vi "Smart_Elevator_TCP.vi"() -> ()   [LabVIEW 2026]
uses:
  Projet_labview/Control 5.ctl
  Projet_labview/Control 6.ctl
  Projet_labview/Control 1.ctl
  <vilib>/Utility/miscctls.llb/LVPositionTypeDef.ctl
panel:
  out "TCP Command Code":i32
  out "Boolean 2":bool
  out "Boolean":bool=TRUE
  out "Numeric 3":i32=2
  out "Numeric 2":i32=1
  out "Numeric":i32
  out "Received Commad":string
  out "?":bool
  out "?":bool
  out "?":picture
  out "Elevator Position":dbl(slide) scale=0.0..2.0 scale format="%#.1g"
  in  "Reset":bool
  out "Curent_STATE":T1
  in  "Quitter":bool
  in  "Urgence_button":bool
  in  "Floor_2":bool
  in  "Floor_1":bool
  in  "RDC":bool
  out "Elevator_STATUS":T3
  # "SMART ELEVATOR CONTROL"
  # "INTELLIGENT LIFT MONITORING & CONTROL"
  # "Elevator_Cabin_Display"
  # "FLOOR 2"
  # "FLOOR 1"
  # "FLOOR G"
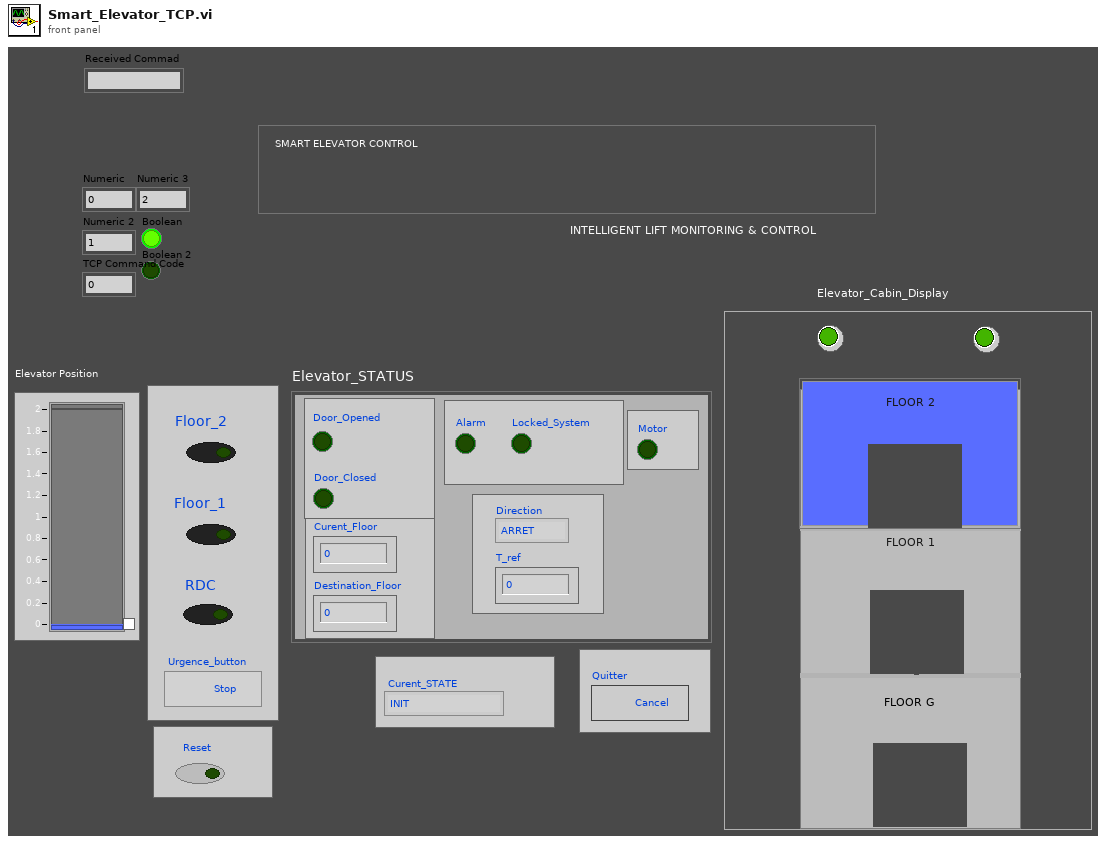
[diagram p1: front panel]
types:
  T1 = typedef "Control 6.ctl" = enum16{"INIT", "ATTENTE", "DEPLACEMENT", "PORTE_OUVERTE", "PORTE_FERMEE", "STOP_URGENT"}
  T2 = typedef "Control 5.ctl" = enum16{"ARRET", "MONTEE", "DESCENTE"}
  T3 = cluster{"Motor":bool, "Door_Opened":bool, "Alarm":bool, "Curent_Floor":i32, "Destination_Floor":i32, "Door_Closed":bool, "T_ref":u32, "Direction":T2, "Locked_System":bool}
  T4 = typedef "Control 1.ctl" = cluster{"Moteur":bool, "Porte_Ouverte":bool, "Alarme":bool, "Position actuelle":i32, "Destination":i32, "Porte_Fermée":bool, "T_ref":u32, "sens":T2, "Systéme_verouillée":bool}
  T5 = typedef "LVPositionTypeDef.ctl" = cluster{"Left":i32, "Top":i32}
  T6 = cluster{"Moteur":bool, "Porte_Ouverte":bool, "Alarme":bool, "Position actuelle":i32, "Destination":i32, "Porte_Fermée":bool, "T_ref":u32, "sens":T2, "Systéme_verouillée":bool}
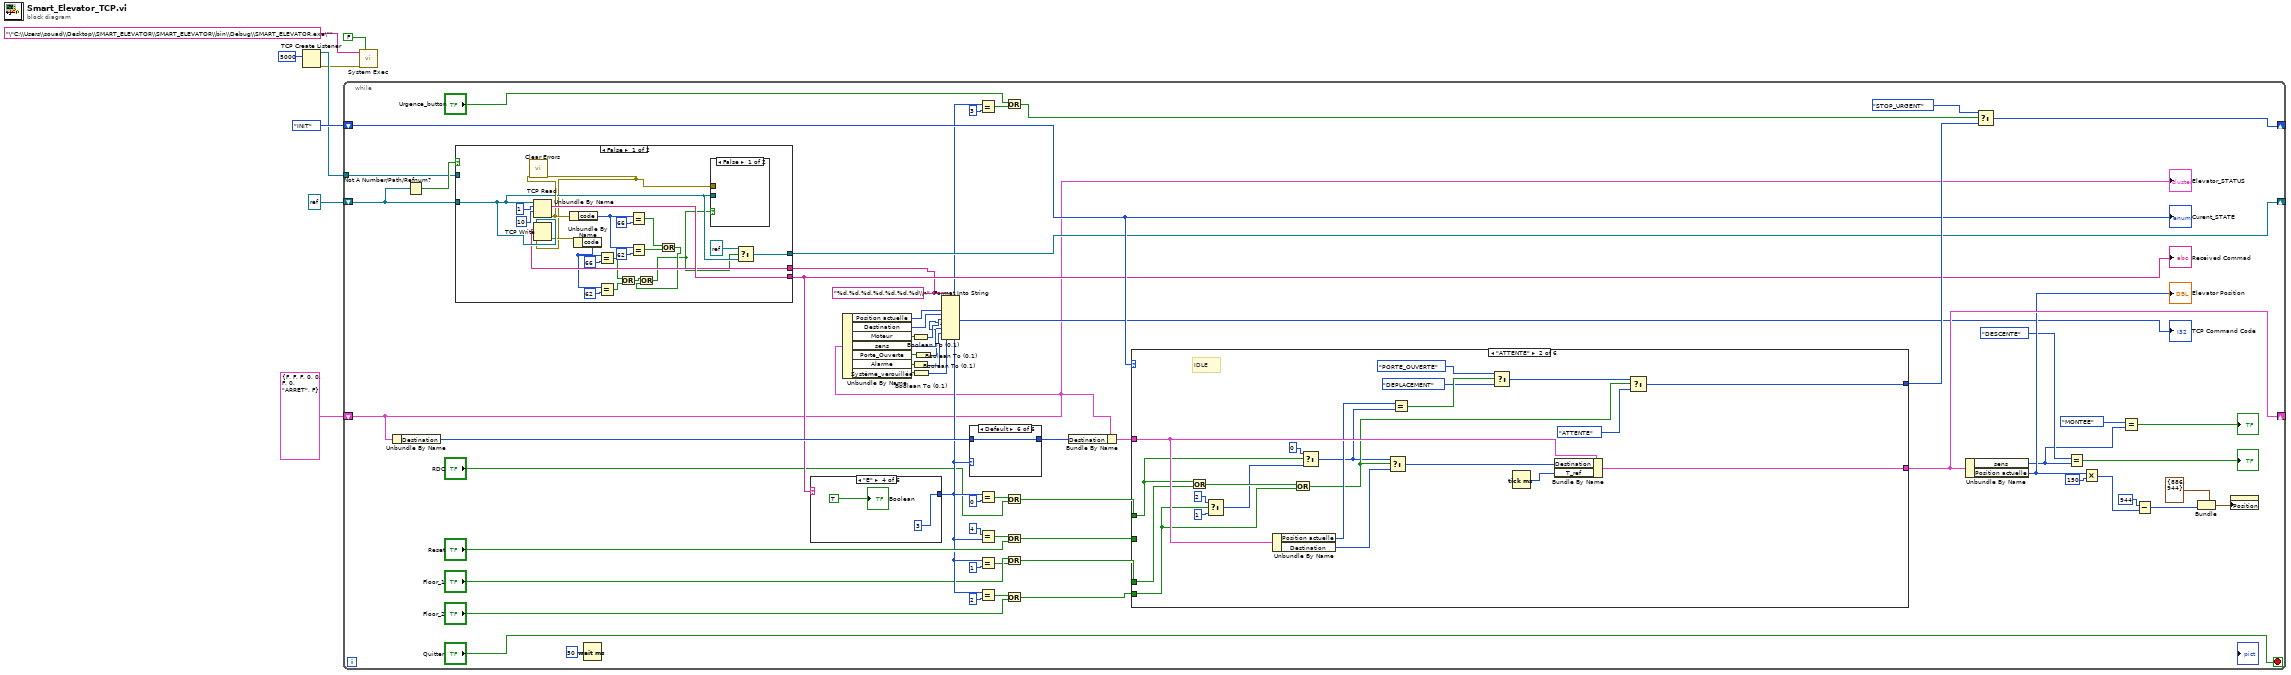
[diagram p0: block diagram]
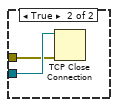
[diagram p2: hidden frame]
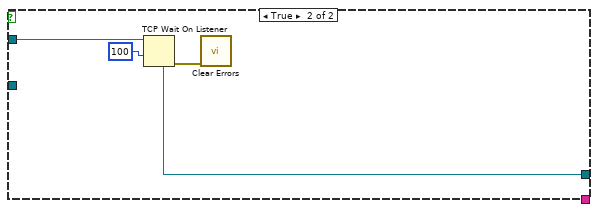
[diagram p3: hidden frame]
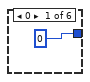
[diagram p4: hidden frame]
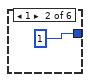
[diagram p5: hidden frame]
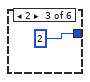
[diagram p6: hidden frame]
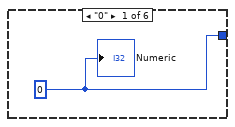
[diagram p9: hidden frame]
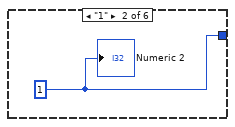
[diagram p10: hidden frame]
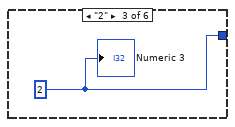
[diagram p11: hidden frame]
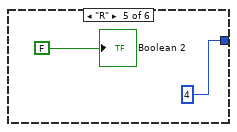
[diagram p12: hidden frame]
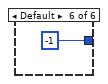
[diagram p13: hidden frame]
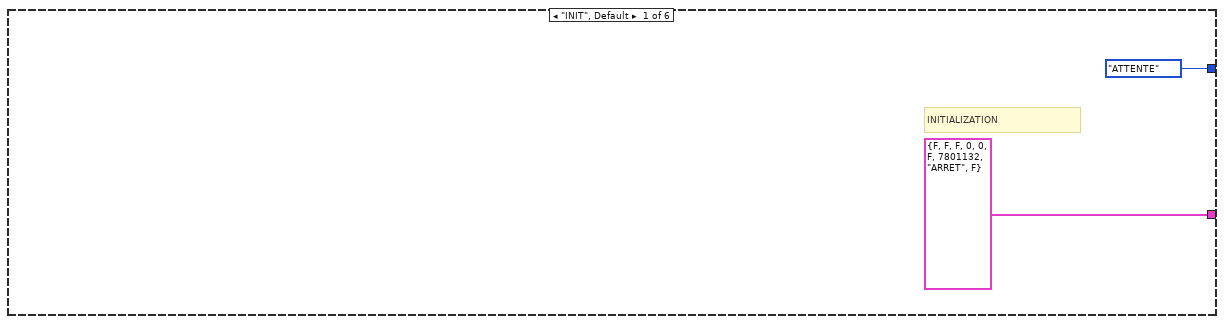
[diagram p14: hidden frame]
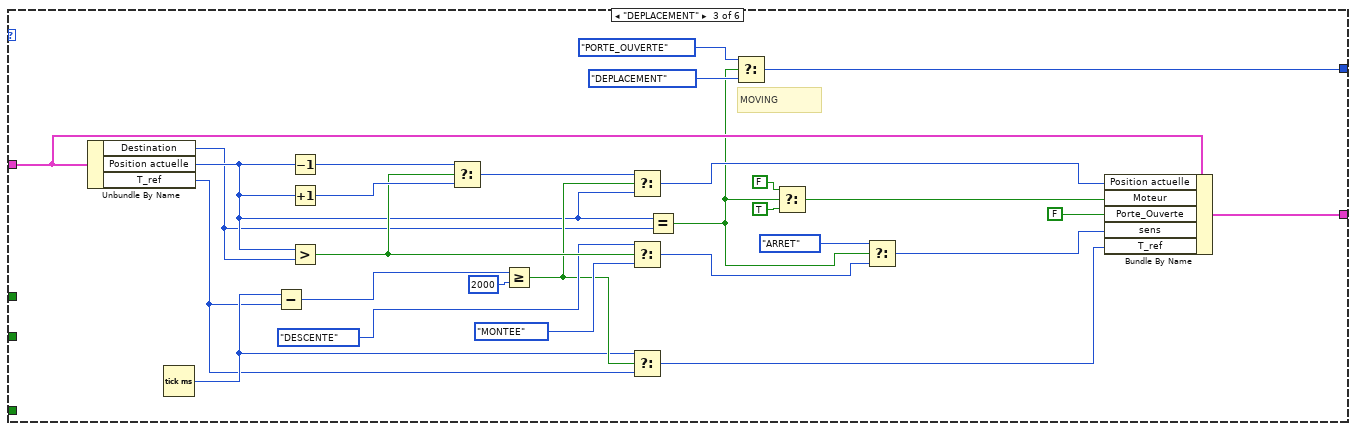
[diagram p15: hidden frame]
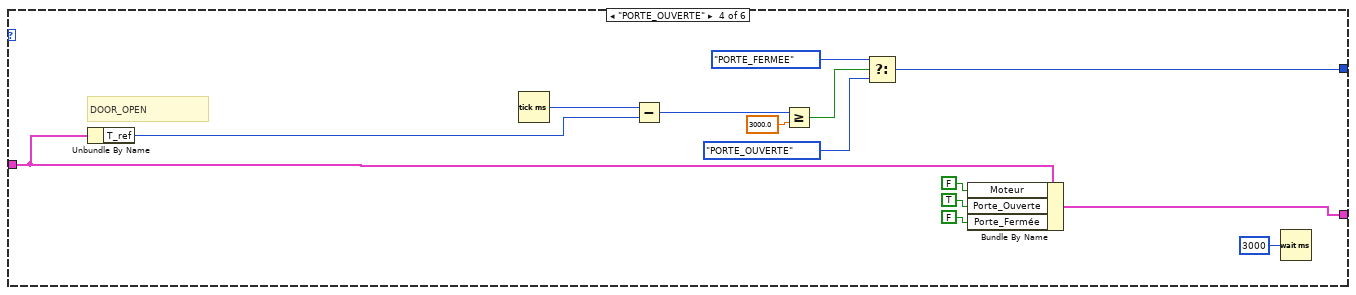
[diagram p16: hidden frame]
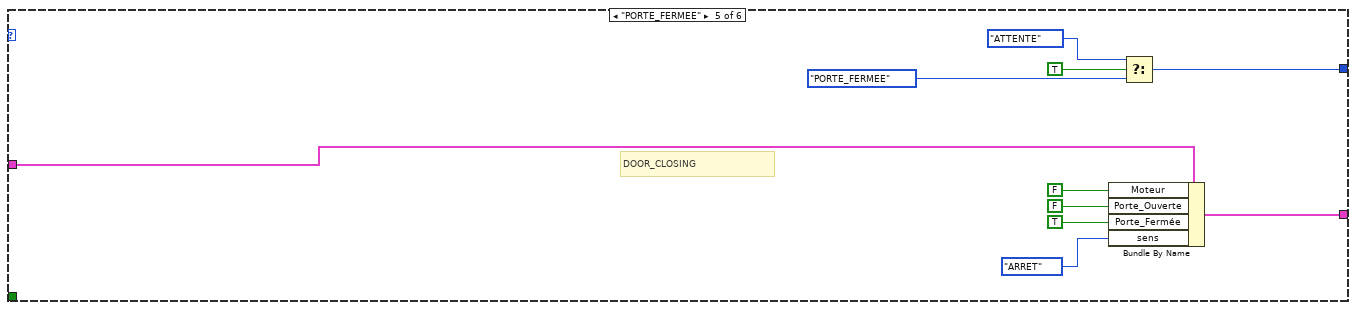
[diagram p17: hidden frame]
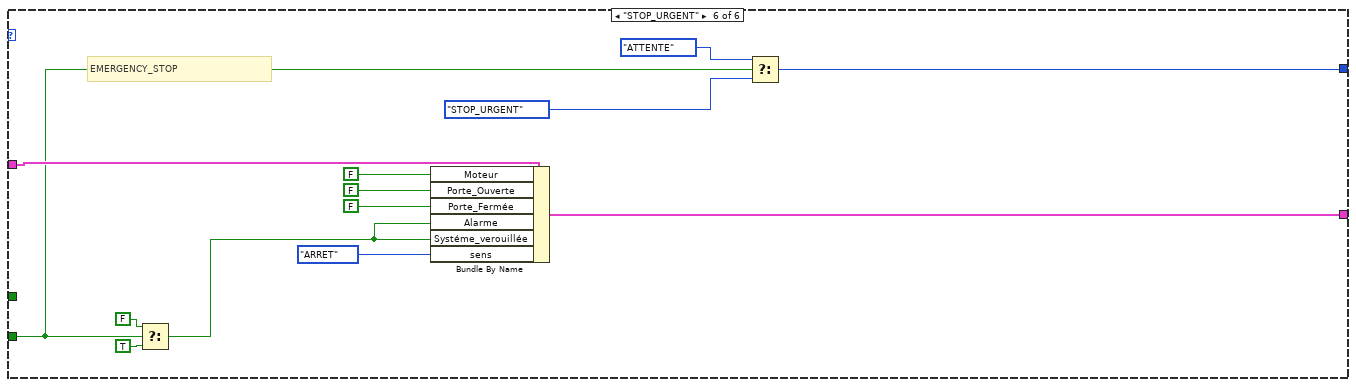
[diagram p18: hidden frame]
diagram:
  n1 = TCP Create Listener(10:u16 5000 ("port")) -> (0:w2:errorcluster, 3:w4:refnum<k5>)  [unwired: 4 in, 1 out]
  n2 = while {
    shift-right: [w66] -> _
    shift-left: Control_6."INIT" ("etat") -> [w64]
    shift-right: [w63] -> _
    shift-left: T4 {"Moteur"=FALSE, "Porte_Ouverte"=FALSE, "Alarme"=FALSE, "Position actuelle"=0, "Destination"=0, "Porte_Fermée"=FALSE, "T_ref"=0, "sens"=enum."ARRET", "Systéme_verouillée"=FALSE} ("Donnees_ASCENCEUR") -> [w21]
    shift-right: [w44] -> _
    shift-left: refnum<k5> refnum ("connection ID") -> [w45]
    tunnel: w4 -> [w46]
    stop <- "Quitter" stop-if-true
    w16 = "%d,%d,%d,%d,%d,%d,%d\\n" ("format string")
    n3 = Unbundle By Name(w21) -> ("Destination"=w49:i32)
    n4 = Not A Number/Path/Refnum?(number/path/refnum=w45) -> (NaN/Path/Refnum?=w47:bool)
    n5 = case shown="False" w47 {
      tunnel: w46 -> [_ w96]
      tunnel: [w83 w97] -> w44
      tunnel: w45 -> [w81 _]
      tunnel: [w90 _] -> w43
      tunnel: w16 -> [w80 _]
      frame False {
        n6 = TCP Read(connection ID=w81, bytes to read=1, 9:10 ("timeout ms (25000)")) -> (data out=w90:string, error out=w82:errorcluster)  [unwired: 2 in, 1 out]
        n7 = call <vilib>:"Clear Errors.vi"("error in (no error)"=w82) -> ("error out"=w70:errorcluster)  [unwired: 5 in, 1 out]
        n8 = TCP Write(connection ID=w81, data in=w80, error in (no error)=w70) -> (error out=w79:errorcluster)  [unwired: 1 in, 2 out]
        n9 = Unbundle By Name(w82) -> ("code"=w88:i32)
        n10 = Unbundle By Name(w79) -> ("code"=w76:i32)
        n11 = Equal?(x=w76, y=66) -> (x = y?=w75:bool)
        n12 = Equal?(x=w76, y=62) -> (x = y?=w74:bool)
        n13 = Or(x=w75, y=w74) -> (x .or. y?=w73:bool)
        n14 = Equal?(x=w88, y=66) -> (x = y?=w86:bool)
        n15 = Equal?(x=w88, y=62) -> (x = y?=w85:bool)
        n16 = Or(x=w86, y=w85) -> (x .or. y?=w72:bool)
        n17 = Or(x=w73, y=w72) -> (x .or. y?=w71:bool)
        n18 = case shown="False" w71 {
          tunnel: w81 -> [_ w94]
          tunnel: w70 -> [_ w93]
          frame False {
          }
          frame True {
            n19 = TCP Close Connection(connection ID=w94, error in (no error)=w93) -> ()  [unwired: 1 in, 2 out]
          }
        }
        n20 = Select(t=refnum<k5> refnum, s=w71, f=w81) -> (s? t:f=w83:refnum<k5>)
      }
      frame True {
        n21 = TCP Wait On Listener(9:100 ("timeout ms (wait forever: -1)"), 11:w96) -> (0:w95:errorcluster, 4:w97:refnum<k5>)  [unwired: 2 in, 3 out]
        n22 = call <vilib>:"Clear Errors.vi"("error in (no error)"=w95) -> ()  [unwired: 5 in, 2 out]
      }
    }
    "Received Commad" <- w43
    n23 = Wait (ms)(milliseconds to wait=u32 50) -> ()  [unwired: 1 out]
    n24 = case shown="\"E\"" w43 {
      tunnel: [w105 w106 w107 3 4 -1] -> w32
      frame "0" {
        w105 = 0
        "Numeric" <- w105
      }
      frame "1" {
        w106 = 1
        "Numeric 2" <- w106
      }
      frame "2" {
        w107 = 2
        "Numeric 3" <- w107
      }
      frame "E" {
        "Boolean" <- TRUE
      }
      frame "R" {
        "Boolean 2" <- FALSE
      }
      frame Default {
      }
    }
    "TCP Command Code" <- w32
    n25 = Unbundle By Name(w21) -> ("Position actuelle"=w15:i32, "Destination"=w14:i32, "Moteur"=w20:bool, "sens"=w12:T2, "Porte_Ouverte"=w19:bool, "Alarme"=w18:bool, "Systéme_verouillée"=w17:bool)
    n26 = Boolean To (0,1)(Boolean=w20) -> (0, 1=w13:i16)
    n27 = Boolean To (0,1)(Boolean=w18) -> (0, 1=w10:i16)
    n28 = Boolean To (0,1)(Boolean=w17) -> (0, 1=w9:i16)
    n29 = Boolean To (0,1)(Boolean=w19) -> (0, 1=w11:i16)
    n30 = Format Into String(format string=w16, w15, w14, w13, w12, w11, w10, w9) -> ()  [unwired: 2 in, 2 out]
    n31 = case shown="Default" w32 {
      tunnel: [0 1 2 w102 w103 w104] -> w50
      tunnel: w49 -> [_ _ _ w102 w103 w104]
      frame 0 {
      }
      frame 1 {
      }
      frame 2 {
      }
      frame 3 {
      }
      frame 4 {
      }
      frame Default {
      }
    }
    n32 = Equal?(x=w32, y=u32 3) -> (x = y?=w36:bool)
    n33 = Equal?(x=w32, y=0) -> (x = y?=w30:bool)
    n34 = Equal?(x=u32 4, y=w32) -> (x = y?=w41:bool)
    n35 = Equal?(x=w32, y=1) -> (x = y?=w27:bool)
    n36 = Equal?(x=w32, y=2) -> (x = y?=w26:bool)
    n37 = Or(x="Urgence_button", y=w36) -> (x .or. y?=w35:bool)
    n38 = Or(x=w30, y="RDC") -> (x .or. y?=w24:bool)
    n39 = Or(x=w41, y="Reset") -> (x .or. y?=w39:bool)
    n40 = Or(x="Floor_1", y=w27) -> (x .or. y?=w23:bool)
    n41 = Or(x=w26, y="Floor_2") -> (x .or. y?=w22:bool)
    n42 = Bundle By Name(cluster=w21, "Destination"=w50) -> (w48:T4)
    n43 = case shown="\"ATTENTE\"" w64 {
      tunnel: w48 -> [_ w131 w164 w169 w188 w201]
      tunnel: [T6 {"Moteur"=FALSE, "Porte_Ouverte"=FALSE, "Alarme"=FALSE, "Position actuelle"=0, "Destination"=0, "Porte_Fermée"=FALSE, "T_ref"=7801132, "sens"=enum."ARRET", "Systéme_verouillée"=FALSE} ("Donnees_ASCENCEUR") w120 w160 w165 w185 w200] -> w63
      tunnel: [Control_6."ATTENTE" ("etat") w124 w151 w170 w181 w195] -> w67
      tunnel: w39 -> [_ _ _ _ _ w192]
      tunnel: w23 -> [_ w123 _ _ _ _]
      tunnel: w24 -> [_ w122 _ _ _ _]
      tunnel: w22 -> [_ w121 _ _ _ _]
      frame "INIT", Default {
        # "INITIALIZATION"
      }
      frame "ATTENTE" {
        # "IDLE"
        n44 = Or(x=w122, y=w123) -> (x .or. y?=w136:bool)
        n45 = Select(t=2, s=w121, f=1) -> (s? t:f=w132:i32)
        n46 = Unbundle By Name(w131) -> ("Position actuelle"=w130:i32, "Destination"=w117:i32)
        n47 = Or(x=w136, y=w121) -> (x .or. y?=w119:bool)
        n48 = Select(t=0, s=w122, f=w132) -> (s? t:f=w118:i32)
        n49 = Select(t=w118, s=w119, f=w117) -> (s? t:f=w116:i32)
        n50 = Equal?(x=w130, y=w118) -> (x = y?=w129:bool)
        n51 = Select(t=Control_6."PORTE_OUVERTE" ("etat"), s=w129, f=Control_6."DEPLACEMENT" ("etat")) -> (s? t:f=w126:T1)
        n52 = Tick Count (ms)() -> (millisecond timer value=w115:u32)
        n53 = Bundle By Name(cluster=w131, "Destination"=w116, "T_ref"=w115) -> (w120:T4)
        n54 = Select(t=w126, s=w119, f=Control_6."ATTENTE" ("etat")) -> (s? t:f=w124:T1)
      }
      frame "DEPLACEMENT" {
        # "MOVING"
        n55 = Unbundle By Name(w164) -> ("Destination"=w138:i32, "Position actuelle"=w139:i32, "T_ref"=w141:u32)
        n56 = Tick Count (ms)() -> (millisecond timer value=w142:u32)
        n57 = Subtract(x=w142, y=w141) -> (x-y=w155:u32)
        n58 = Decrement(x=w139) -> (x-1=w157:i32)
        n59 = Increment(x=w139) -> (x+1=w158:i32)
        n60 = Greater?(x=w139, y=w138) -> (0:w150:bool)
        n61 = Select(t=w157, s=w150, f=w158) -> (s? t:f=w137:i32)
        n62 = Greater Or Equal?(x=w155, y=u32 2000) -> (x >= y?=w143:bool)
        n63 = Select(t=w137, s=w143, f=w139) -> (s? t:f=w154:i32)
        n64 = Select(t=Control_5."DESCENTE" ("sens"), s=w150, f=Control_5."MONTEE" ("sens")) -> (s? t:f=w145:T2)
        n65 = Select(t=w142, s=w143, f=w141) -> (s? t:f=w140:u32)
        n66 = Equal?(x=w139, y=w138) -> (x = y?=w147:bool)
        n67 = Select(t=Control_6."PORTE_OUVERTE" ("etat"), s=w147, f=Control_6."DEPLACEMENT" ("etat")) -> (s? t:f=w151:T1)
        n68 = Select(t=FALSE, s=w147, f=TRUE) -> (s? t:f=w161:bool)
        n69 = Select(t=Control_5."ARRET" ("sens"), s=w147, f=w145) -> (s? t:f=w144:T2)
        n70 = Bundle By Name(cluster=w164, "Position actuelle"=w154, "Moteur"=w161, "Porte_Ouverte"=FALSE, "sens"=w144, "T_ref"=w140) -> (w160:T4)
      }
      frame "PORTE_OUVERTE" {
        # "DOOR_OPEN"
        n71 = Unbundle By Name(w169) -> ("T_ref"=w176:u32)
        n72 = Tick Count (ms)() -> (millisecond timer value=w177:u32)
        n73 = Subtract(x=w177, y=w176) -> (x-y=w174:u32)
        n74 = Greater Or Equal?(x=w174, y=3000.0) -> (x >= y?=w173:bool)
        n75 = Select(t=Control_6."PORTE_FERMEE" ("etat"), s=w173, f=Control_6."PORTE_OUVERTE" ("etat")) -> (s? t:f=w170:T1)
        n76 = Bundle By Name(cluster=w169, "Moteur"=FALSE, "Porte_Ouverte"=TRUE, "Porte_Fermée"=FALSE) -> (w165:T4)
        n77 = Wait (ms)(milliseconds to wait=u32 3000) -> ()  [unwired: 1 out]
      }
      frame "PORTE_FERMEE" {
        # "DOOR_CLOSING"
        n78 = Bundle By Name(cluster=w188, "Moteur"=FALSE, "Porte_Ouverte"=FALSE, "Porte_Fermée"=TRUE ("Porte_Ouverte"), "sens"=Control_5."ARRET") -> (w185:T4)
        n79 = Select(t=Control_6."ATTENTE" ("etat"), s=TRUE, f=Control_6."PORTE_FERMEE" ("etat")) -> (s? t:f=w181:T1)
      }
      frame "STOP_URGENT" {
        # "EMERGENCY_STOP"
        n80 = Select(t=FALSE, s=w192, f=TRUE) -> (s? t:f=w189:bool)
        n81 = Bundle By Name(cluster=w201, "Moteur"=FALSE, "Porte_Ouverte"=FALSE, "Porte_Fermée"=FALSE ("Porte_Ouverte"), "Alarme"=w189, "Systéme_verouillée"=w189, "sens"=Control_5."ARRET") -> (w200:T4)
        n82 = Select(t=Control_6."ATTENTE" ("etat"), s=w192, f=Control_6."STOP_URGENT" ("etat")) -> (s? t:f=w195:T1)
      }
    }
    n83 = Unbundle By Name(w63) -> ("sens"=w53:T2, "Position actuelle"=w62:i32)
    "Elevator Position" <- w62
    n84 = Select(t=Control_6."STOP_URGENT" ("etat"), s=w35, f=w67) -> (s? t:f=w66:T1)
    n85 = Equal?(x=Control_5."DESCENTE" ("sens"), y=w53) -> (x = y?=→"?":bool)
    n86 = Multiply(x=w62, y=150) -> (x*y=w60:i32)
    n87 = Equal?(x=Control_5."MONTEE" ("sens"), y=w53) -> (x = y?=→"?":bool)
    n88 = Subtract(x=944, y=w60) -> (x-y=w58:i32)
    n89 = Bundle(cluster=T5 {"Left"=886, "Top"=944} ("Position"), "Top"=w58) -> (w56:T5)  [unwired: 1 in]
    n90 = property class="Pict"("Position"=w56) -> ()  [unwired: 2 in, 2 out]
    "Curent_STATE" <- w64
    "Elevator_STATUS" <- w21
  }
  n91 = call <vilib>:"System Exec.vi"("wait until completion? (T)"=FALSE, "error in (no error)"=w2, "command line"="\"C:\\Users\\souad\\Desktop\\SMART_ELEVATOR\\SMART_ELEVATOR\\bin\\Debug\\SMART_ELEVATOR.exe\"") -> ()  [unwired: 5 in, 4 out]
